vi "New UTF-8 Path.vi"(7 "Input Encoding (ANSI)":T1, 9 "error in":errorcluster, 10 "LabVIEW Path":path) -> (1 "error out":errorcluster, 2 "UTF-8 Path":refnum<class "UTF-8 Path.lvclass">)   [LabVIEW 2020, in "G-Unicode.lvlib" / "UTF-8 Path.lvclass"]
doc: "Initializes a new UTF-8 Path. <b>Path</b> can be ANSI, UTF-8, or UTF-16LE encoded. The path encoding is determined automatically when <b>Encoding</b> is set to Auto, or explicitly when set to ANSI, UTF-8 UTF-16LE, or UTF-16BE.\n\nNote that automatic encoding detection isn't 100% accurate, and it is recommended to set the encoding explicitly if it is known.\n\n<b>ANSI</b> will be encoded as UTF-8 using the local codepage.\n<b>UTF-8</b> will be unchanged.\n<b>UTF-16LE</b> and <b>UTF-16BE</b> will be converted to UTF-8."
uses:
  UTF-8 Path.lvclass
  Unicode/Controls/String Encoding.ctl
  UTF-8 Path.lvclass/UTF-8 Path.ctl
  Private/Conversion/Text to UTF-8.vi
  Private/Conversion/Polymorphic VIs/Text to UTF-8 (LabVIEW String).vi
  Private/Conversion/Encoded UTF-8 String to Encoded UTF-16LE String.vi
  Private/Conversion/UTF-8 to Text.vi
  Private/Conversion/Polymorphic VIs/UTF-8 to Text (LabVIEW String).vi
  Private/Conversion/Encoded UTF-16LE String to Encoded UTF-8 String.vi
  Unicode/SubVIs/UTF-16 Byte Swap.vi
  Unicode/Prepend BOM.vi
  Unicode/SubVIs/Byte Order Marks.vi
  Unicode/Detect BOM.vi
  Unicode/Detect String Encoding.vi
  G-Unicode.lvlib
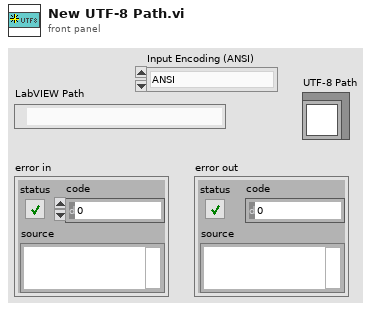
[diagram p1: front panel]
types:
  T1 = typedef "G-Unicode.lvlib/String Encoding.ctl" = enum16{"ANSI", "UTF-8", "UTF-16LE", "UTF-16BE", "Unknown"}
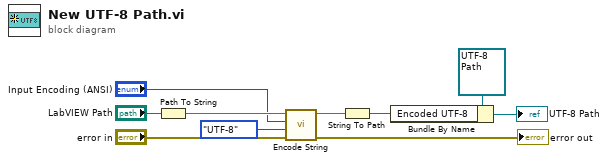
[diagram p0: block diagram]
diagram:
  n1 = Path To String(path="LabVIEW Path") -> (string=w6:string)
  n2 = call "Encode String.vi"("error in"="error in", "Output Encoding (UTF-16LE)"=String_Encoding."UTF-8", "Input Encoding (ANSI)"="Input Encoding (ANSI)", "String in"=w6) -> ("error out"=→"error out":errorcluster, "String out"=w2:string)  [unwired: 6 in]
  n3 = String To Path(string=w2) -> (path=w7:path)
  n4 = Bundle By Name(cluster=refnum<class "UTF-8 Path.lvclass"> refnum ("UTF-8 Path"), "Encoded UTF-8"=w7) -> (→"UTF-8 Path":refnum<class "UTF-8 Path.lvclass">)
